vi "Message alerte AL reg.vi"(2 "Données alarmes":string[](array[string]), 3 "alarmes 1COM reg":string[](array[string]), 4 "Noms voies regs sélect acqui 1 COM":string, 5 "Message entrée":string) -> (1 "Message sortie":string)   [LabVIEW 2022 SP3]
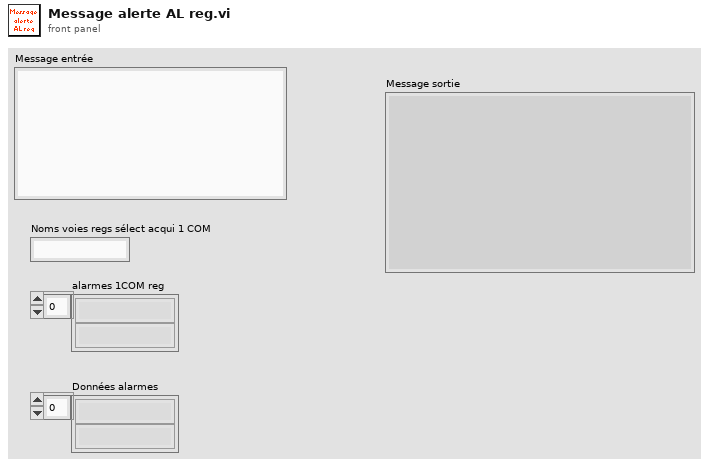
[diagram p1: front panel]
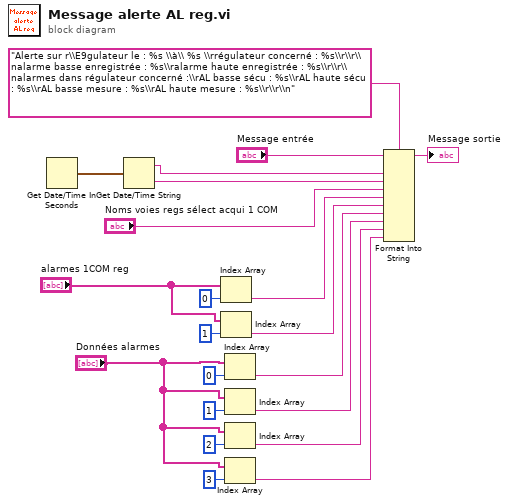
[diagram p0: block diagram]
diagram:
  n1 = Get Date/Time In Seconds() -> (seconds since 1Jan1904=w21:timestamp)
  n2 = Get Date/Time String(seconds (now)=w21) -> (date string=w20:string, time string=w19:string)  [unwired: 2 in]
  n3 = Index Array(array="alarmes 1COM reg", index=0 ("indice")) -> (element=w13:string)
  n4 = Index Array(array="alarmes 1COM reg", index=1 ("indice")) -> (element=w10:string)
  n5 = Index Array(array="Données alarmes", index=0 ("indice")) -> (element=w5:string)
  n6 = Index Array(array="Données alarmes", index=1 ("indice")) -> (element=w4:string)
  n7 = Index Array(array="Données alarmes", index=2 ("indice")) -> (element=w2:string)
  n8 = Index Array(array="Données alarmes", index=3 ("indice")) -> (element=w1:string)
  n9 = Format Into String(format string="Alerte sur r\\E9gulateur le : %s \\à\\ %s \\rrégulateur concerné : %s\\r\\r\\nalarme basse enregistrée : %s\\ralarme haute enregistrée : %s\\r\\r\\nalarmes dans régulateur concerné :\\rAL basse sécu : %s\\rAL haute sécu : %s\\rAL basse mesure : %s\\rAL haute mesure : %s\\r\\r\\n" ("chaîne de format"), initial string="Message entrée", w20, w19, "Noms voies regs sélect acqui 1 COM", w13, w10, w5, w4, w2, w1) -> (resulting string=→"Message sortie":string)  [unwired: 1 in, 1 out]
